vi "lvmcp_indexmode.vi"() -> ()   [LabVIEW 2026]
panel:
  out "error out":errorcluster
  in  "mode":i32
  in  "reference":refnum<vi>
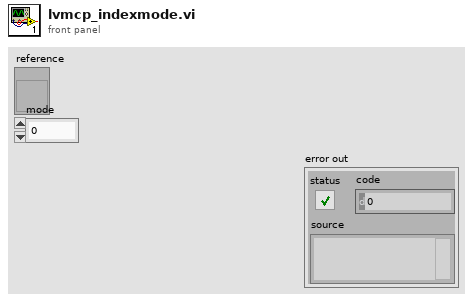
[diagram p1: front panel]
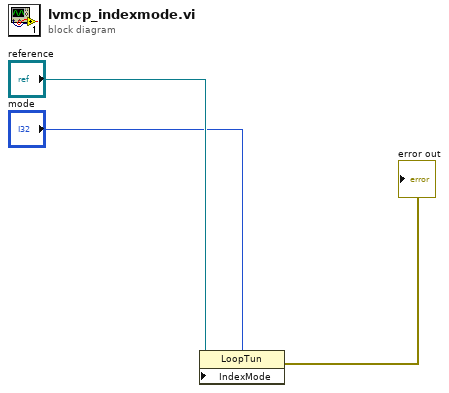
[diagram p0: block diagram]
diagram:
  n1 = property class="LoopTun"(reference="reference", "IndexMode"="mode") -> (error out=→"error out":errorcluster)  [unwired: 1 in, 1 out]
